vi "Add Client.vi"(6 "Service Name":string, 8 "error in (no error)":errorcluster, 9 "Client ID":string, 10 "WebSocket Connection":refnum<k5>, 11 "WebSocket Service Actor in":refnum<class "WebSocket Service.lvclass">) -> (0 "error out":errorcluster, 3 "WebSocket Service Actor out":refnum<class "WebSocket Service.lvclass">)   [LabVIEW 2021, in "WebSocket Actors.lvlib" / "WebSocket Service.lvclass"]
doc: "The WebSocket server has successfully completed the handshake and accepted client connection. This method starts the WebSocket Connection actor that will handle the communication to this particular client connected to this service"
uses:
  WebSocket Service.lvclass
  C:/Program Files/National Instruments/LabVIEW 2021/vi.lib/ActorFramework/Actor/Actor.lvclass
  WebSocket Connection/WebSocket Connection.lvclass
  WebSocket Service Messages/WebSocket Service Connection Handler Msg/WebSocket Service Connection Handler Msg.lvclass
  C:/Projects/WebSocket-Actor/WebSocket Actor/Abstract Messages/WebSocket Connection Handler Msg/WebSocket Connection Handler Msg.lvclass
  <vilib>/ActorFramework/Actor/Actor.lvclass/Actor.ctl
  <vilib>/ActorFramework/Message Enqueuer/Message Enqueuer.lvclass/Message Enqueuer.ctl
  WebSocket Service.lvclass/WebSocket Service.ctl
  WebSocket Connection/WebSocket Connection.lvclass/WebSocket Connection.ctl
  WebSocket Connection/properties/Write Timeout.vi
  WebSocket Connection/Write Keepalive.vi
  WebSocket Connection/properties/Write WebSocket Connection.vi
  WebSocket Connection/properties/Write WebSocket Data Handler.vi
  WebSocket Connection/properties/Write Peer ID.vi
  <vilib>/ActorFramework/Message Enqueuer/Init from Existing Queue.vi
  <vilib>/ActorFramework/Message Enqueuer/Message Enqueuer.lvclass
  <vilib>/ActorFramework/Actor/Actor.lvclass
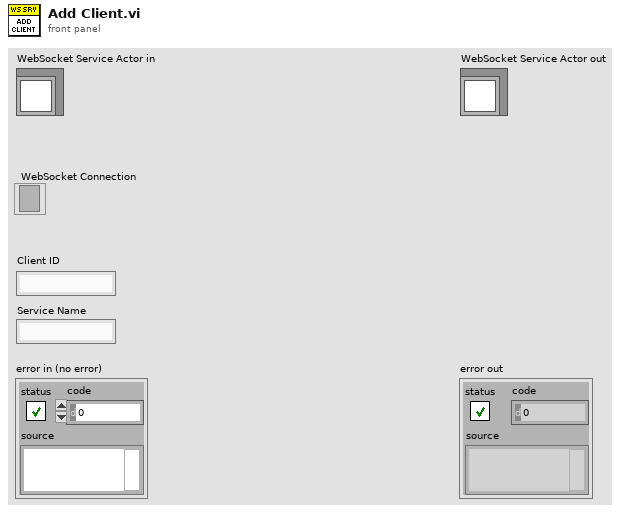
[diagram p1: front panel]
types:
  T1 = typedef "WebSocket Actors.lvlib/WebSocket Connection.lvclass/Keepalive.ctl" = cluster{"Enabled":bool, "Ping Interval (ms)":u32, "Ping Timeout (ms)":u32}
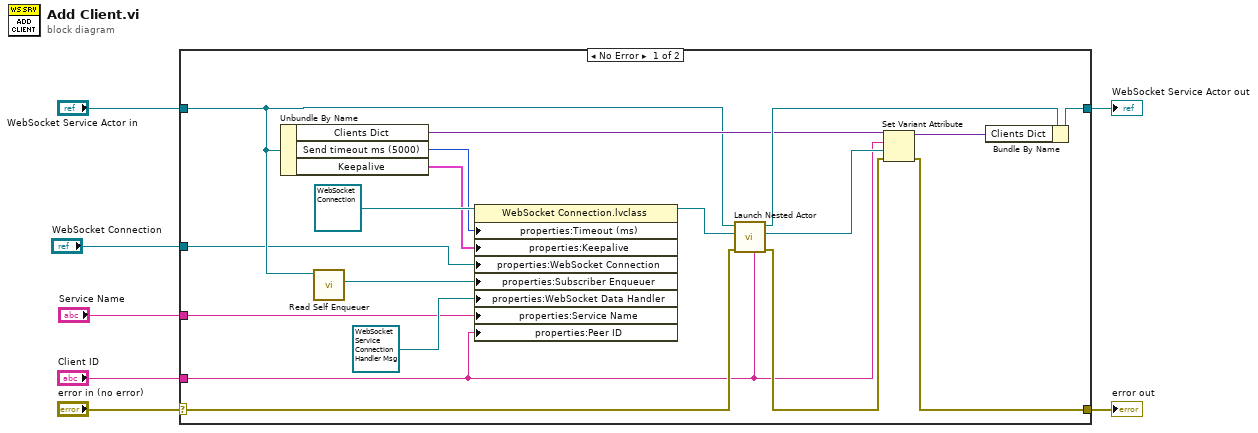
[diagram p0: block diagram]
diagram:
  n1 = case shown="No Error" "error in (no error)" {
    selector: "error in (no error)" -> [w23 w27]
    tunnel: [w16 w27] -> w6
    tunnel: [w21 w26] -> w4
    tunnel: "WebSocket Service Actor in" -> [w14 w26]
    tunnel: "WebSocket Connection" -> [w13 _]
    tunnel: "Client ID" -> [w12 _]
    tunnel: "Service Name" -> [w10 _]
    frame No Error {
      n2 = Unbundle By Name(w14) -> ("Clients Dict"=w20:variant, "Send timeout ms (5000)"=w9:i32, "Keepalive"=w8:T1)
      n3 = call <vilib>:"Read Self Enqueuer.vi"("Actor"=w14) -> ("Self Enqueuer"=w11:refnum<class "Message Enqueuer.lvclass">)  [unwired: 10 in]
      n4 = property class="WebSocket Connection.lvclass"(reference=refnum<class "WebSocket Connection.lvclass"> refnum ("WebSocket Connection.lvclass"), "properties:Timeout (ms)"=w9, "properties:Keepalive"=w8, "properties:WebSocket Connection"=w13, "properties:Subscriber Enqueuer"=w11, "properties:WebSocket Data Handler"=refnum<class "WebSocket Service Connection Handler Msg.lvclass"> refnum ("WebSocket Actors.lvlib:WebSocket Service Data Handler Msg.lvclass"), "properties:Service Name"=w10, "properties:Peer ID"=w12) -> (reference out=w25:refnum<class "WebSocket Connection.lvclass">)  [unwired: 1 in, 1 out]
      n5 = call <vilib>:"Launch Nested Actor.vi"("Debug Alias"=w12, "error in (no error)"=w23, "Nested Actor"=w25, "Caller Actor in"=w14) -> ("error out"=w17:errorcluster, "Nested Actor's Enqueuer"=w18:refnum<class "Message Enqueuer.lvclass">, "Caller Actor out"=w24:refnum<class "WebSocket Service.lvclass">)  [unwired: 5 in]
      n6 = Set Variant Attribute(Variant=w20, name=w12, value=w18, error in=w17) -> (Variant out=w19:variant, error out=w16:errorcluster)  [unwired: 1 out]
      n7 = Bundle By Name(cluster=w24, "Clients Dict"=w19) -> (w21:refnum<class "WebSocket Service.lvclass">)
    }
    frame Error {
    }
  }
  "error out" <- w6
  "WebSocket Service Actor out" <- w4
